vi "Manage Server Attribute.vi"(0 "All Interfaces Dict in":variant, 2 "Specific Interface Dict in":variant, 3 "Message Enqueuer in":refnum<class "Message Enqueuer.lvclass">, 4 "Listener Settings":T1, 5 "error in (no error)":errorcluster, 8 "Is \"All Interface\" Server":bool, 9 "Action":enum16{"Set", "Get", "Delete"}(ring)) -> (14 "All Interfaces Dict out":variant, 16 "Specific Interface Dict out":variant, 17 "Message Enqueuer out":refnum<class "Message Enqueuer.lvclass">, 19 "error out":errorcluster)   [LabVIEW 2016, in "WebSocket Actors.lvlib" / "WebSocket Server Manager.lvclass"]
uses:
  WebSocket Server Manager.lvclass
  <vilib>/ActorFramework/Message Enqueuer/Message Enqueuer.lvclass
  WebSocket Server/typedefs/Listener Settings.ctl
  WebSocket Server/WebSocket Server.lvclass
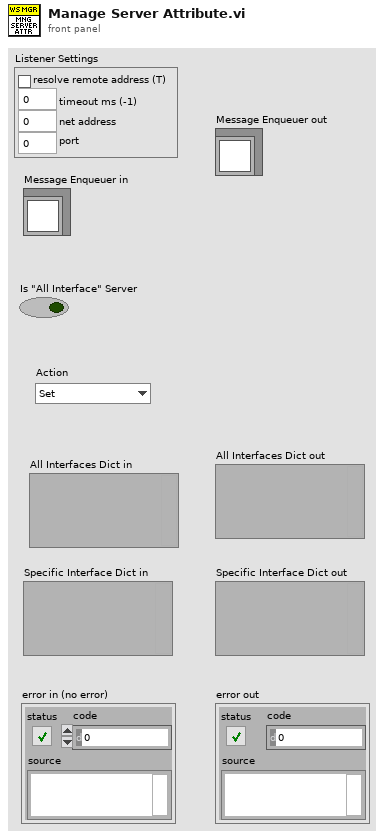
[diagram p1: front panel]
types:
  T1 = typedef "WebSocket Actors.lvlib/WebSocket Server.lvclass/Listener Settings.ctl" = cluster{"resolve remote address (T)":bool, "timeout ms (-1)":i32, "net address":u32, "port":u16}
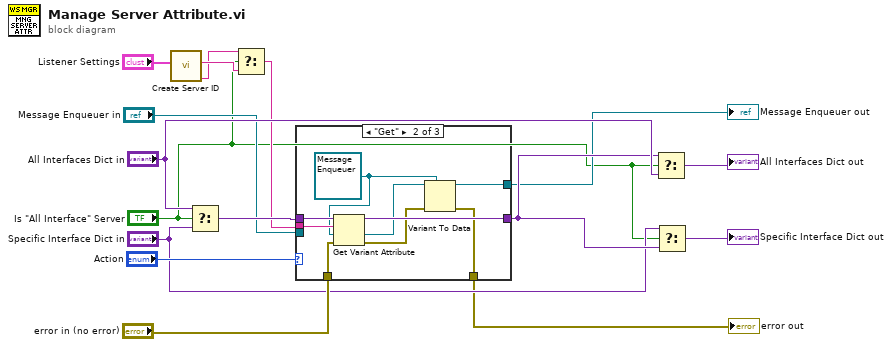
[diagram p0: block diagram]
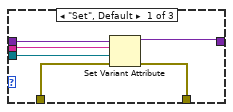
[diagram p2: hidden frame]
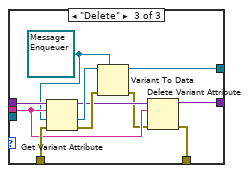
[diagram p3: hidden frame]
diagram:
  n1 = call "Create Server ID.vi"("Listener Settings"="Listener Settings") -> ("Port String"=w1:string, "Server URI"=w3:string)  [unwired: 7 in, 1 out]
  n2 = Select(t="All Interfaces Dict in", s="Is \"All Interface\" Server", f="Specific Interface Dict in") -> (s? t:f=w13:variant)
  n3 = Select(t=w1, s="Is \"All Interface\" Server", f=w3) -> (s? t:f=w4:string)
  n4 = case shown="\"Get\"" "Action" {
    tunnel: w13 -> [w21 w31 w36]
    tunnel: [w20 w30 w41] -> w10
    tunnel: "error in (no error)" -> [w22 w29 w38]
    tunnel: [w19 w25 w42] -> w6
    tunnel: w4 -> [w18 w28 w37]
    tunnel: "Message Enqueuer in" -> [w17 _ _]
    tunnel: [_ w24 w34] -> w5
    frame "Set", Default {
      n5 = Set Variant Attribute(Variant=w21, name=w18, value=w17, error in=w22) -> (Variant out=w20:variant, error out=w19:errorcluster)  [unwired: 1 out]
    }
    frame "Get" {
      w23 = refnum<class "Message Enqueuer.lvclass"> refnum ("Nested Actor's Enqueuer")
      n6 = Get Variant Attribute(Variant=w31, name=w28, default value (empty Variant)=w23, error in=w29) -> (duplicate Variant=w30:variant, value=w26:refnum<class "Message Enqueuer.lvclass">, error out=w27:errorcluster)  [unwired: 1 out]
      n7 = Variant To Data(error in=w27, type=w23, Variant=w26) -> (data=w24:refnum<class "Message Enqueuer.lvclass">, error out=w25:errorcluster)
    }
    frame "Delete" {
      w32 = refnum<class "Message Enqueuer.lvclass"> refnum ("Nested Actor's Enqueuer")
      n8 = Get Variant Attribute(Variant=w36, name=w37, default value (empty Variant)=w32, error in=w38) -> (duplicate Variant=w35:variant, value=w40:refnum<class "Message Enqueuer.lvclass">, error out=w39:errorcluster)  [unwired: 1 out]
      n9 = Variant To Data(error in=w39, type=w32, Variant=w40) -> (data=w34:refnum<class "Message Enqueuer.lvclass">, error out=w33:errorcluster)
      n10 = Delete Variant Attribute(4:w33, 6:w37, 7:w35) -> (0:w42:errorcluster, 3:w41:variant)  [unwired: 1 out]
    }
  }
  "Message Enqueuer out" <- w5
  "error out" <- w6
  n11 = Select(t=w10, s="Is \"All Interface\" Server", f="All Interfaces Dict in") -> (s? t:f=→"All Interfaces Dict out":variant)
  n12 = Select(t="Specific Interface Dict in", s="Is \"All Interface\" Server", f=w10) -> (s? t:f=→"Specific Interface Dict out":variant)
